vi "VIH Utility - VISRV - Get Datatype Terminal Icon - Build Datatype ID.vi"(11 "Datatype":variant) -> (3 "Type ID":u64 format="%.0x")   [LabVIEW 2014]
doc: "::: VI Helpeks :::\nCopyright (c) 2000-2026 Konstantin Shifershteyn. All rights reserved."
panel:
  # "5400000000"
  # "VI Helpeks\nCopyright (c) 2012-2026 Konstantin Shifershteyn"
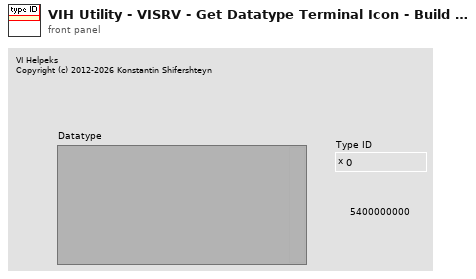
[diagram p1: front panel]
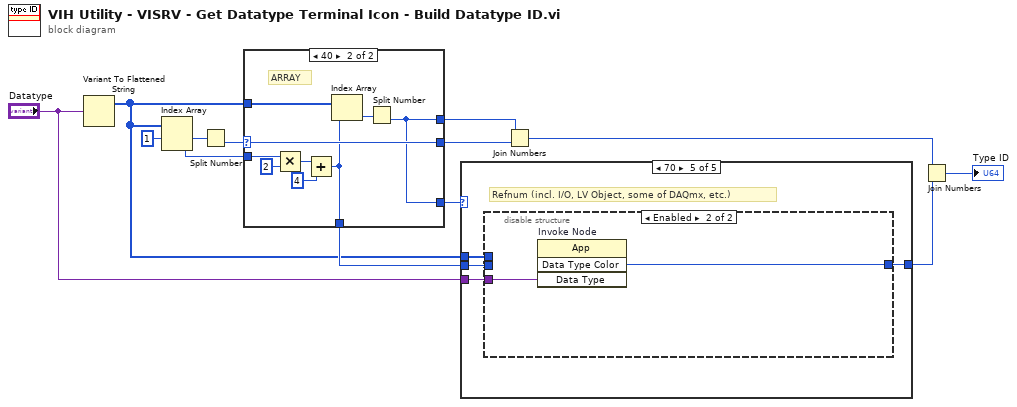
[diagram p0: block diagram]
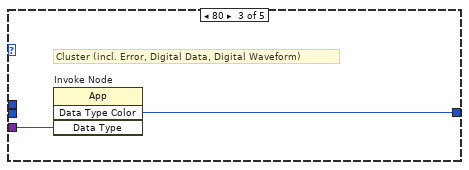
[diagram p4: hidden frame]
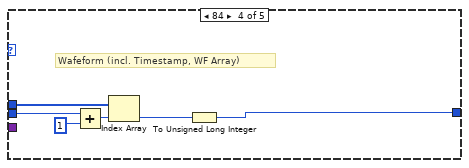
[diagram p5: hidden frame]
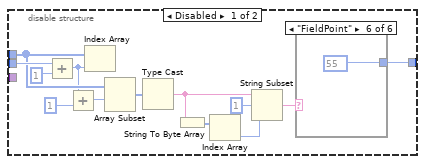
[diagram p6: hidden frame]
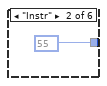
[diagram p8: hidden frame]
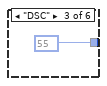
[diagram p9: hidden frame]
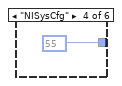
[diagram p10: hidden frame]
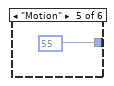
[diagram p11: hidden frame]
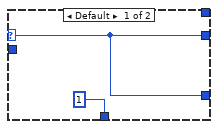
[diagram p12: hidden frame]
diagram:
  n1 = Variant To Flattened String(Variant="Datatype") -> (1:w1:i16[])  [unwired: 1 out]
  n2 = Index Array(array=w1, index #1=1 ("index")) -> (element #1=w9:i16, element #2=w10:i16)  [unwired: 1 in]
  n3 = Split Number(x=w9) -> (lo(x)=w11:u8)  [unwired: 1 out]
  n4 = case shown="40" w11 {
    selector: w11 -> [w15 w18]
    tunnel: w10 -> [_ w21]
    tunnel: w1 -> [_ w20]
    tunnel: [_ w17] -> w12
    tunnel: [w15 w18] -> w13
    tunnel: [w15 w17] -> w6
    tunnel: [1 w16] -> w2
    frame Default {
    }
    frame 64 {
      # "ARRAY"
      n5 = Multiply(x=w21, y=i16 2) -> (x*y=w23:i16)
      n6 = Add(x=w23, y=i16 4) -> (x+y=w16:i16)
      n7 = Index Array(array=w20, index=w16) -> (element=w19:i16)
      n8 = Split Number(x=w19) -> (lo(x)=w17:u8)  [unwired: 1 out]
    }
  }
  n9 = case shown="70" w6 {
    tunnel: "Datatype" -> [_ _ w26 _ w33]
    tunnel: [_ _ w25 w27 w34] -> w5
    tunnel: w1 -> [_ _ _ w32 w35]
    tunnel: w2 -> [_ _ _ w29 w36]
    frame Default {
    }
    frame 55 {
      # "DAQ, DAQmx (not all)"
    }
    frame 80 {
      # "Cluster (incl. Error, Digital Data, Digital Waveform)"
      n10 = invoke on="Invoke Node" class="App" method="Data Type Color"("Data Type"=w26) -> ("Data Type Color"=w25:u32)  [unwired: 3 in, 3 out]
    }
    frame 84 {
      # "Wafeform (incl. Timestamp, WF Array)"
      n11 = Add(x=w29, y=1 ("index")) -> (x+y=w31:i32)
      n12 = Index Array(array=w32, index=w31) -> (element=w28:i16)
      n13 = To Unsigned Long Integer(number=w28) -> (unsigned 32bit integer=w27:u32)
    }
    frame 112 {
      # "Refnum (incl. I/O, LV Object, some of DAQmx, etc.)"
      n14 = disable-structure shown="Enabled" {
        disable-tunnel: w36 -> [w48 _]
        disable-tunnel: w35 -> [w47 _]
        disable-tunnel: [w39 w55] -> w34
        disable-tunnel: w33 -> [_ w56]
        frame Disabled {
          n15 = Add(x=w48, y=1 ("index")) -> (x+y=w45:i32)
          n16 = Add(x=w45, y=1) -> (x+y=w46:i32)
          n17 = Index Array(array=w47, index=w45) -> ()  [unwired: 1 out]
          n18 = Array Subset(array=w47, index=w46) -> (w43:i16[])  [unwired: 1 in]
          n19 = Type Cast(x=w43) -> (*(type *) &x=w37:string)  [unwired: 1 in]
          n20 = String To Byte Array(string=w37) -> (unsigned byte array=w38:u8[])
          n21 = Index Array(array=w38) -> (element=w41:u8)  [unwired: 1 in]
          n22 = String Subset(string=w37, offset (0)=1, length (rest)=w41) -> (substring=w40:string)
          n23 = case shown="\"FieldPoint\"" w40 {
            tunnel: [_ u32 55 ("Data Type Color") u32 55 ("Data Type Color") u32 55 ("Data Type Color") u32 55 ("Data Type Color") u32 55 ("Data Type Color")] -> w39
            frame Default {
            }
            frame "Instr" {
            }
            frame "DSC" {
            }
            frame "NISysCfg" {
            }
            frame "Motion" {
            }
            frame "FieldPoint" {
            }
          }
        }
        frame Enabled {
          n24 = invoke on="Invoke Node" class="App" method="Data Type Color"("Data Type"=w56) -> ("Data Type Color"=w55:u32)  [unwired: 3 in, 3 out]
        }
      }
    }
  }
  n25 = Join Numbers(hi=w12, lo=w13) -> ((hi.lo)=w4:u16)
  n26 = Join Numbers(hi=w4, lo=w5) -> ((hi.lo)=→"Type ID":u64)
